vi "set Trigger Level.vi"(8 "error in (no error)":errorcluster, 10 "Trigger Level (dBm)":dbl, 11 "FSV-40N in":refnum<class "FSV-40N.lvclass">) -> (0 "error out":errorcluster, 3 "FSV-40N out":refnum<class "FSV-40N.lvclass">)   [LabVIEW 2023, in "Spectrum Analyzer.lvlib" / "FSV-40N.lvclass"]
uses:
  FSV-40N.lvclass
  FSV-40N.lvclass/FSV-40N.ctl
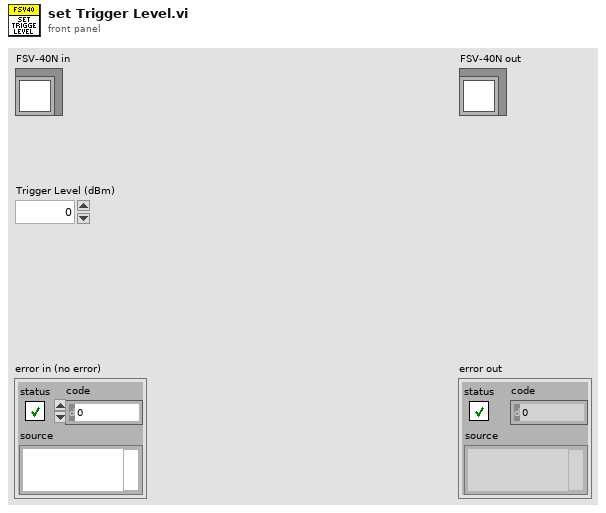
[diagram p1: front panel]
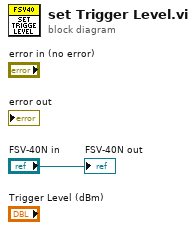
[diagram p0: block diagram]
diagram:
  "FSV-40N out" <- "FSV-40N in"
